vi "Find NI-SWITCH Custom Device.vi"   [LabVIEW 2020, in "NI-SWITCH Scripting.lvlib"]
doc: "Returns the NI-SWITCH custom device(s) under the specified target."
uses:
  NI-SWITCH Scripting.lvlib
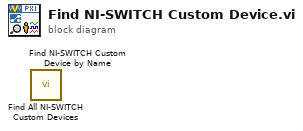
[diagram p0: block diagram]
diagram:
  n1 = call "Find All NI-SWITCH Custom Devices.vi"() -> ()  [unwired: 9 in, 3 out]
  n2 = call "Find NI-SWITCH Custom Device by Name.vi"() -> ()  [unwired: 9 in, 3 out]
